vi "Polymorphic.vi"   [LabVIEW 2020]
doc: "1421114"
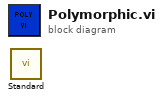
[diagram p0: block diagram]
diagram:
  n1 = call "Standard.vi"() -> ()  [unwired: 9 in, 3 out]
